vi "openbci_reset_hw_32bit.vi"(8 "error in (no error)":errorcluster, 11 "OBCI dev in":T1={"COM port"="", "n_ch (8)"=enum."8 Channels", "delay_tx"=50}) -> (0 "error out":errorcluster, 2 "reset_str":string, 3 "OBCI dev out":T1={"COM port"="", "n_ch (8)"=enum."8 Channels", "delay_tx"=50})   [LabVIEW 2013]
doc: "OpenBCI to reset hardware in case of 32bit board"
uses:
  Control Def/openbci_device.ctl
  Control Def/channel_count.ctl
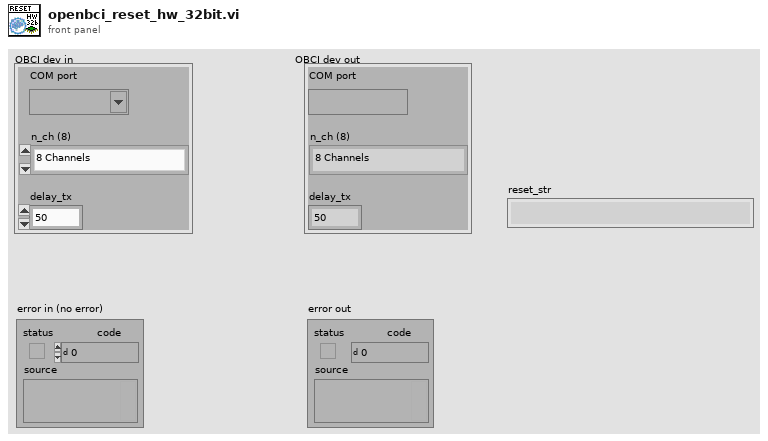
[diagram p1: front panel]
types:
  T1 = typedef "openbci_device.ctl" = cluster{"COM port":refnum<visa-resource-name>, "n_ch (8)":T2, "delay_tx":u32}
  T2 = typedef "channel_count.ctl" = enum16{"8 Channels", "16 Channels"}
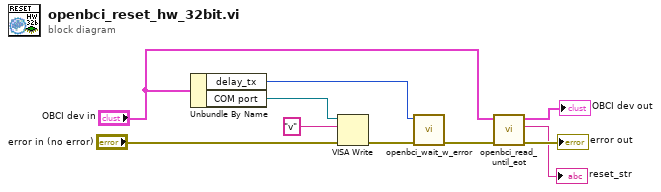
[diagram p0: block diagram]
diagram:
  n1 = Unbundle By Name("OBCI dev in") -> ("delay_tx"=w6:u32, "COM port"=w8:refnum<visa-resource-name>)
  n2 = VISA Write(VISA resource name=w8, write buffer="v", error in (no error)="error in (no error)") -> (error out=w7:errorcluster)  [unwired: 2 out]
  n3 = call "openbci_wait_w_error.vi"("error in (no error)"=w7, "milliseconds to wait"=w6) -> ("error out"=w5:errorcluster)  [unwired: 9 in]
  n4 = call "openbci_read_until_eot.vi"("error in"=w5, "OBCI dev in"="OBCI dev in") -> ("error out"=→"error out":errorcluster, "string"=→"reset_str":string, "OBCI dev out"=→"OBCI dev out":T1)  [unwired: 7 in]
